vi "Configure Module.vi"(8 "error in (no error)":errorcluster, 10 "IOV ref in":variant, 11 "Module Template in":refnum<class "9209.lvclass">) -> (0 "error out":errorcluster, 2 "IOV ref out":variant, 3 "Module Template out":refnum<class "9209.lvclass">)   [LabVIEW 2020, in "Modules.lvlib" / "9209.lvclass"]
uses:
  9209.lvclass
  <resource>/objmgr/cRIO.rc
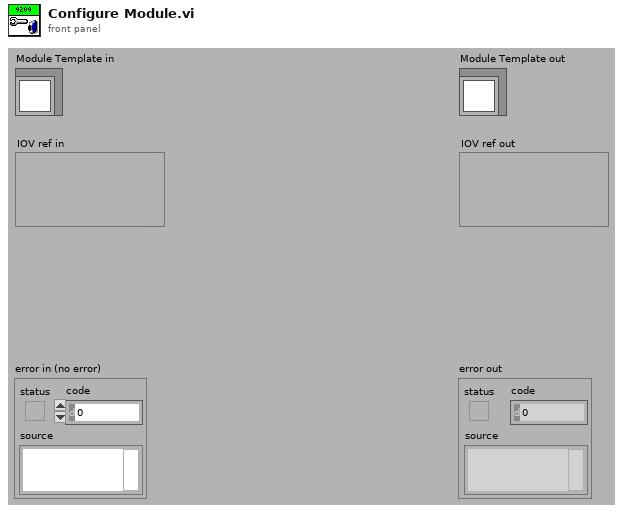
[diagram p1: front panel]
types:
  T1 = typedef "Modules.lvlib/9209.lvclass/Channel Settings.ctl" = T2[]
  T2 = typedef "Modules.lvlib/9209.lvclass/Terminal mode.ctl" = enum16{"RSE", "DIFF"}
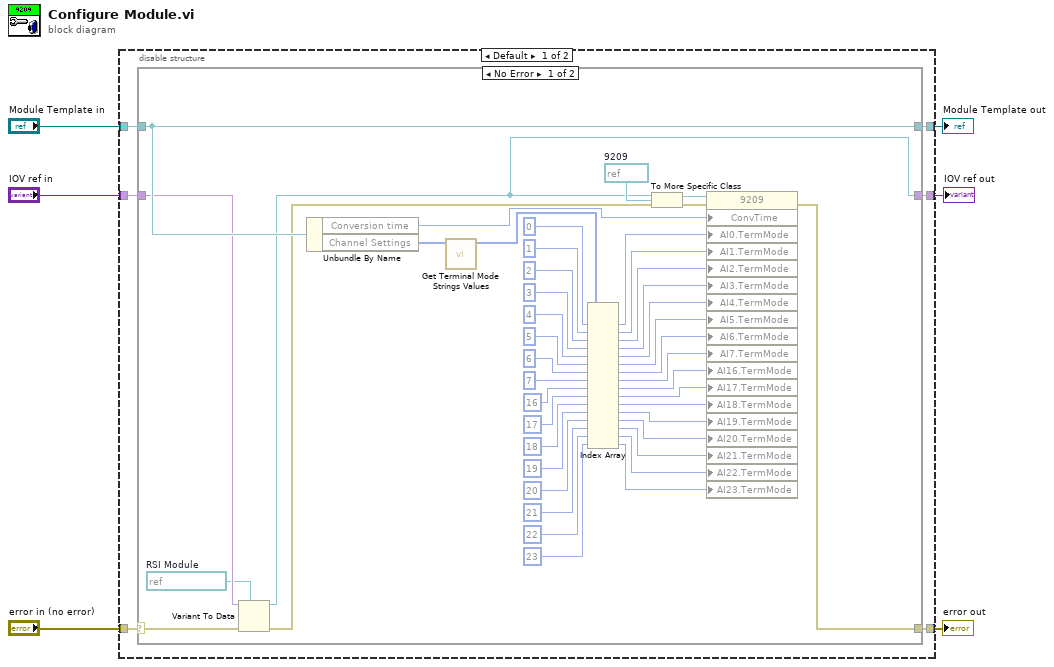
[diagram p0: block diagram]
diagram:
  n1 = disable-structure shown="Default" {
    disable-tunnel: "error in (no error)" -> [w12 w63]
    disable-tunnel: [w11 w63] -> w5
    disable-tunnel: "Module Template in" -> [w10 w61]
    disable-tunnel: [w9 w61] -> w3
    disable-tunnel: "IOV ref in" -> [w8 w62]
    disable-tunnel: [w7 w62] -> w1
    frame condition #0 {
      n2 = case shown="No Error" w12 {
        selector: w12 -> [w54 w60]
        tunnel: [w57 w60] -> w11
        tunnel: [w55 w59] -> w9
        tunnel: w10 -> [w55 w59]
        tunnel: w8 -> [w15 w58]
        tunnel: [w14 w58] -> w7
        frame No Error {
          w13 = refnum<k21> refnum  # RSI Module
          w53 = refnum<k21> refnum  # 9209
          n3 = Variant To Data(error in=w54, type=w13, Variant=w15) -> (data=w14:refnum<k21>, error out=w16:errorcluster)
          n4 = Unbundle By Name(w55) -> ("Conversion time"=w56:u32, "Channel Settings"=w18:T1)
          n5 = call "Get Terminal Mode Strings Values.vi"("Terminal Mode Display Values"=w18) -> ("Terminal Mode RSI Values"=w17:u32[])  [unwired: 10 in]
          n6 = Index Array(array=w17, index #1=0 ("index"), index #2=1 ("index"), index #3=2 ("index"), index #4=3 ("index"), index #5=4 ("index"), index #6=5 ("index"), index #7=6 ("index"), index #8=7 ("index"), index #9=16 ("index"), index #10=17 ("index"), index #11=18 ("index"), index #12=19 ("index"), index #13=20 ("index"), index #14=21 ("index"), index #15=22 ("index"), index #16=23 ("index")) -> (element #1=w34:u32, element #2=w33:u32, element #3=w32:u32, element #4=w31:u32, element #5=w30:u32, element #6=w29:u32, element #7=w28:u32, element #8=w27:u32, element #9=w26:u32, element #10=w25:u32, element #11=w24:u32, element #12=w23:u32, element #13=w22:u32, element #14=w21:u32, element #15=w19:u32, element #16=w20:u32)
          n7 = To More Specific Class(target class=w53, reference=w14, error in=w16) -> (specific class reference=w52:refnum<k21>, error out=w51:errorcluster)
          n8 = property class="9209"(reference=w52, error in=w51, "ConvTime"=w56, "AI0.TermMode"=w34, "AI1.TermMode"=w33, "AI2.TermMode"=w32, "AI3.TermMode"=w31, "AI4.TermMode"=w30, "AI5.TermMode"=w29, "AI6.TermMode"=w28, "AI7.TermMode"=w27, "AI16.TermMode"=w26, "AI17.TermMode"=w25, "AI18.TermMode"=w24, "AI19.TermMode"=w23, "AI20.TermMode"=w22, "AI21.TermMode"=w21, "AI22.TermMode"=w19, "AI23.TermMode"=w20) -> (error out=w57:errorcluster)  [unwired: 1 out]
        }
        frame Error {
        }
      }
    }
    frame condition #1 (active) {
    }
  }
  "error out" <- w5
  "Module Template out" <- w3
  "IOV ref out" <- w1
